vi "Target must be a directory--error.vi"() -> (0 "error out":errorcluster)   [LabVIEW 2026]
doc: "This error signalizes that the specified target for a file manager operation must be a directory and it is not."
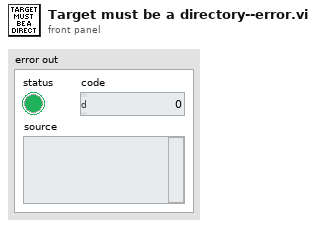
[diagram p1: front panel]
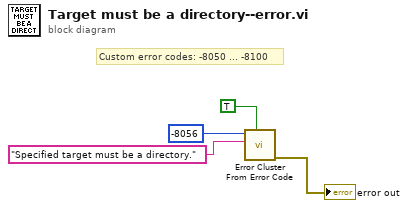
[diagram p0: block diagram]
diagram:
  # "Custom error codes: -8050 ... -8100"
  n1 = call <vilib>:"Error Cluster From Error Code.vi"("show call chain? (False)"=TRUE, "error message (\"\")"="Specified target must be a directory." ("error message (\"\")"), "error code (0)"=-8056) -> ("error out"=→"error out":errorcluster)  [unwired: 6 in]
